vi "sqlite Connect.vi"(6 "QuotesOnTable":bool, 8 "error in (no error)":errorcluster, 10 "Connection String":string, 11 "SQLiteJDPMapper":refnum<class "Mapper.lvclass">) -> (0 "error out":errorcluster, 3 "SqlMapper out":refnum<class "SqlMapper.lvclass">)   [LabVIEW 2020, in "ORM_sqlite_jdp.lvlib" / "DBC.lvclass"]
uses:
  DBC.lvclass
  <vilib>/Viviota/shared/ORM.lvlibp/SqlMapper/SqlMapper.lvclass
  PGJDPMapper/Mapper.lvclass
  C:/Program Files (x86)/National Instruments/LabVIEW 2020/vi.lib/Viviota/shared/ORM.lvlibp/SqlMapper/SqlMapper.lvclass
  DBC.lvclass/DBC.ctl
  C:/Program Files (x86)/National Instruments/LabVIEW 2020/vi.lib/Viviota/shared/ORM.lvlibp/DbConnection/DbConnection.lvclass
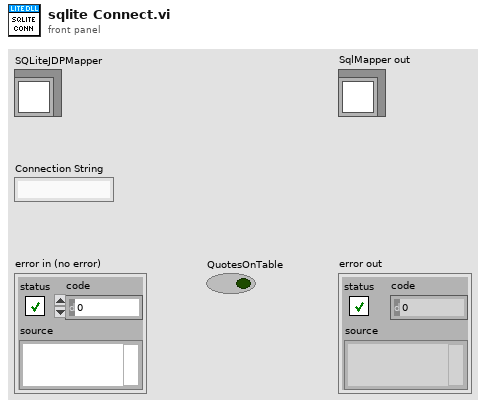
[diagram p1: front panel]
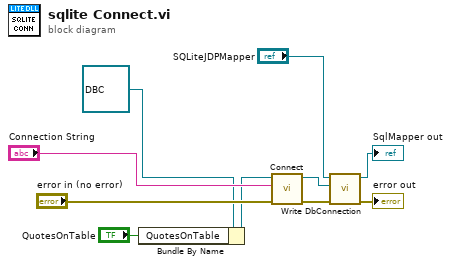
[diagram p0: block diagram]
diagram:
  n1 = Bundle By Name(cluster=refnum<class "DBC.lvclass"> refnum ("PostgresqlConnection.lvclass"), "QuotesOnTable"="QuotesOnTable") -> (w3:refnum<class "DBC.lvclass">)
  n2 = call-dynamic "Connect.vi"("error in (no error)"="error in (no error)", "Connection String"="Connection String", "PostgresqlConnection in"=w3) -> ("error out"=w7:errorcluster, "PostgresqlConnection out"=w5:refnum<class "DBC.lvclass">)  [unwired: 7 in]
  n3 = call <vilib>:"Write DbConnection.vi"("error in (no error)"=w7, "Dapper.lvlib:DbConnection.lvclass"=w5, "SqlMapper in"="SQLiteJDPMapper") -> ("error out"=→"error out":errorcluster, "SqlMapper out"=→"SqlMapper out":refnum<class "Mapper.lvclass">)  [unwired: 7 in]
